vi "lvmcp_conpane.vi"() -> ()   [LabVIEW 2015]
panel:
  out "Controls[]":refnum<vi>[](array[refnum])
  out "error out":errorcluster
  in  "reference":refnum<vi>
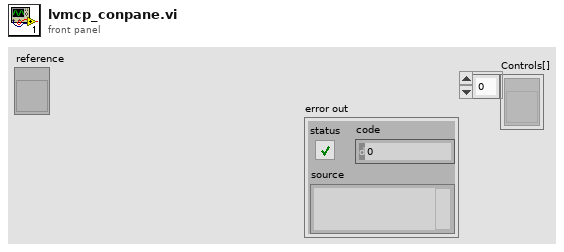
[diagram p1: front panel]
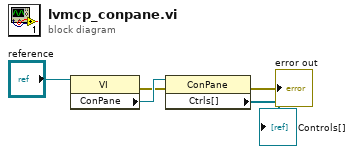
[diagram p0: block diagram]
diagram:
  n1 = property class="VI"(reference="reference") -> (error out=w3:errorcluster, "ConPane"=w4:refnum<vi>)  [unwired: 1 in, 1 out]
  n2 = property class="ConPane"(reference=w4, error in=w3) -> (error out=→"error out":errorcluster, "Ctrls[]"=→"Controls[]":refnum<vi>[])  [unwired: 1 out]
